vi "CIVI Error Query.vi"(8 "error in":errorcluster, 11 "VISA Session in":refnum<visa-resource-name>="TCPIP0::127.0.0.1::5025::SOCKET") -> (0 "error out":errorcluster, 2 "SCPI Error Code":i32, 3 "VISA Session out":refnum<visa-resource-name>)   [LabVIEW 2026]
doc: "Queries SYST:ERR? and parses one entry from the error queue\nfor the current connection.\nReturns the SCPI error code separately.\nA nonzero SCPI code produces LabVIEW error 5000,\nwith the full response in source.\nCommunication and parsing errors take precedence.\nDoes not drain the entire error queue.\nCheck error out before interpreting the numeric SCPI code."
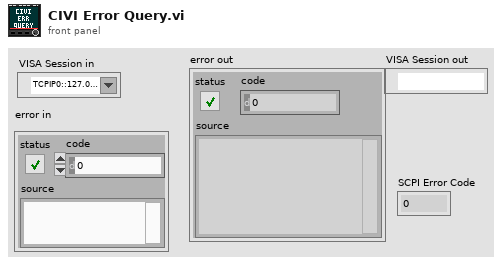
[diagram p1: front panel]
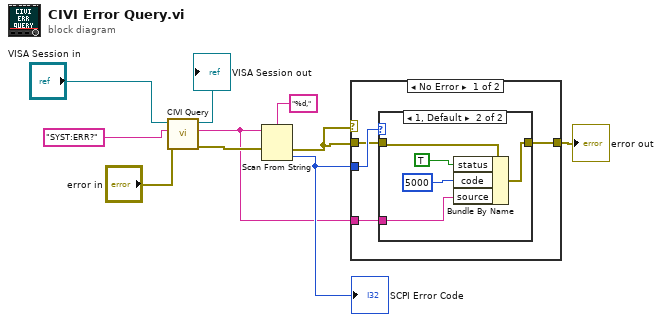
[diagram p0: block diagram]
diagram:
  n1 = call "CIVI Query.vi"("error in"="error in", "write buffer"="SYST:ERR?", "VISA Session in"="VISA Session in") -> ("error out"=w5:errorcluster, "read buffer"=w1:string, "VISA Session out"=→"VISA Session out":refnum<visa-resource-name>)  [unwired: 6 in]
  n2 = Scan From String(format string="%d,", input string=w1, error in=w5) -> (error out=w3:errorcluster, output 1=w2:i32)  [unwired: 2 in, 2 out]
  "SCPI Error Code" <- w2
  n3 = case shown="No Error" w3 {
    tunnel: [w12 w21] -> w4
    tunnel: w3 -> [w13 w21]
    tunnel: w2 -> [w14 _]
    tunnel: w1 -> [w11 _]
    frame No Error {
      n4 = case shown="1, Default" w14 {
        tunnel: w13 -> [w15 w20]
        tunnel: [w15 w19] -> w12
        tunnel: w11 -> [_ w18]
        frame 0 {
        }
        frame 1, Default {
          n5 = Bundle By Name(cluster=w20, "status"=TRUE, "code"=5000, "source"=w18) -> (w19:errorcluster)
        }
      }
    }
    frame Error {
    }
  }
  "error out" <- w4
